vi "LEYBOLD.vi"() -> ()   [LabVIEW 2022 SP3]
uses:
  Enum/Enum p1.ctl
  <vilib>/Instr/_visa.llb/VISA Flush IO Buffer Mask.ctl
  Variables globales/Variable glob Leybold.vi
  Variables globales/Variable glob generale.vi
  <vilib>/Instr/_visa.llb/VISA Configure Serial Port (Instr).vi
panel:
  out "Données Leybold":string[](array[string])
  out "VISA":refnum<visa-resource-name>[](array[refnum])
  out "Chaine lue :":string
  # "Dialogue avec les CENTER-ONE"
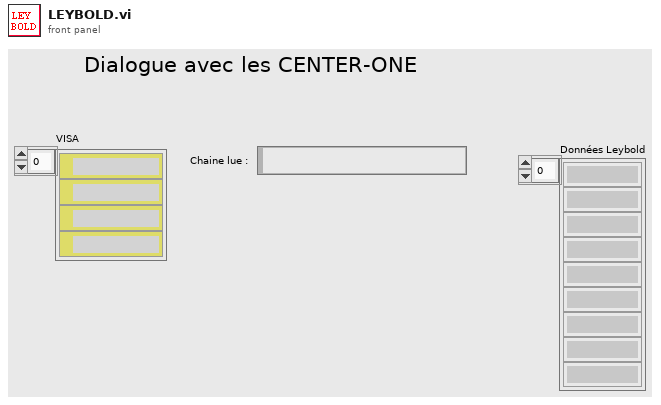
[diagram p1: front panel]
types:
  T1 = typedef "Enum p1.ctl" = enum16{"init", "Lecture pour vider buffer", "écriture val pres", "lecture ACK", "écriture ENQ", "lecture pres", "traitement chaine", "erreur"}
  T2 = typedef "VISA Flush IO Buffer Mask.ctl" = u16
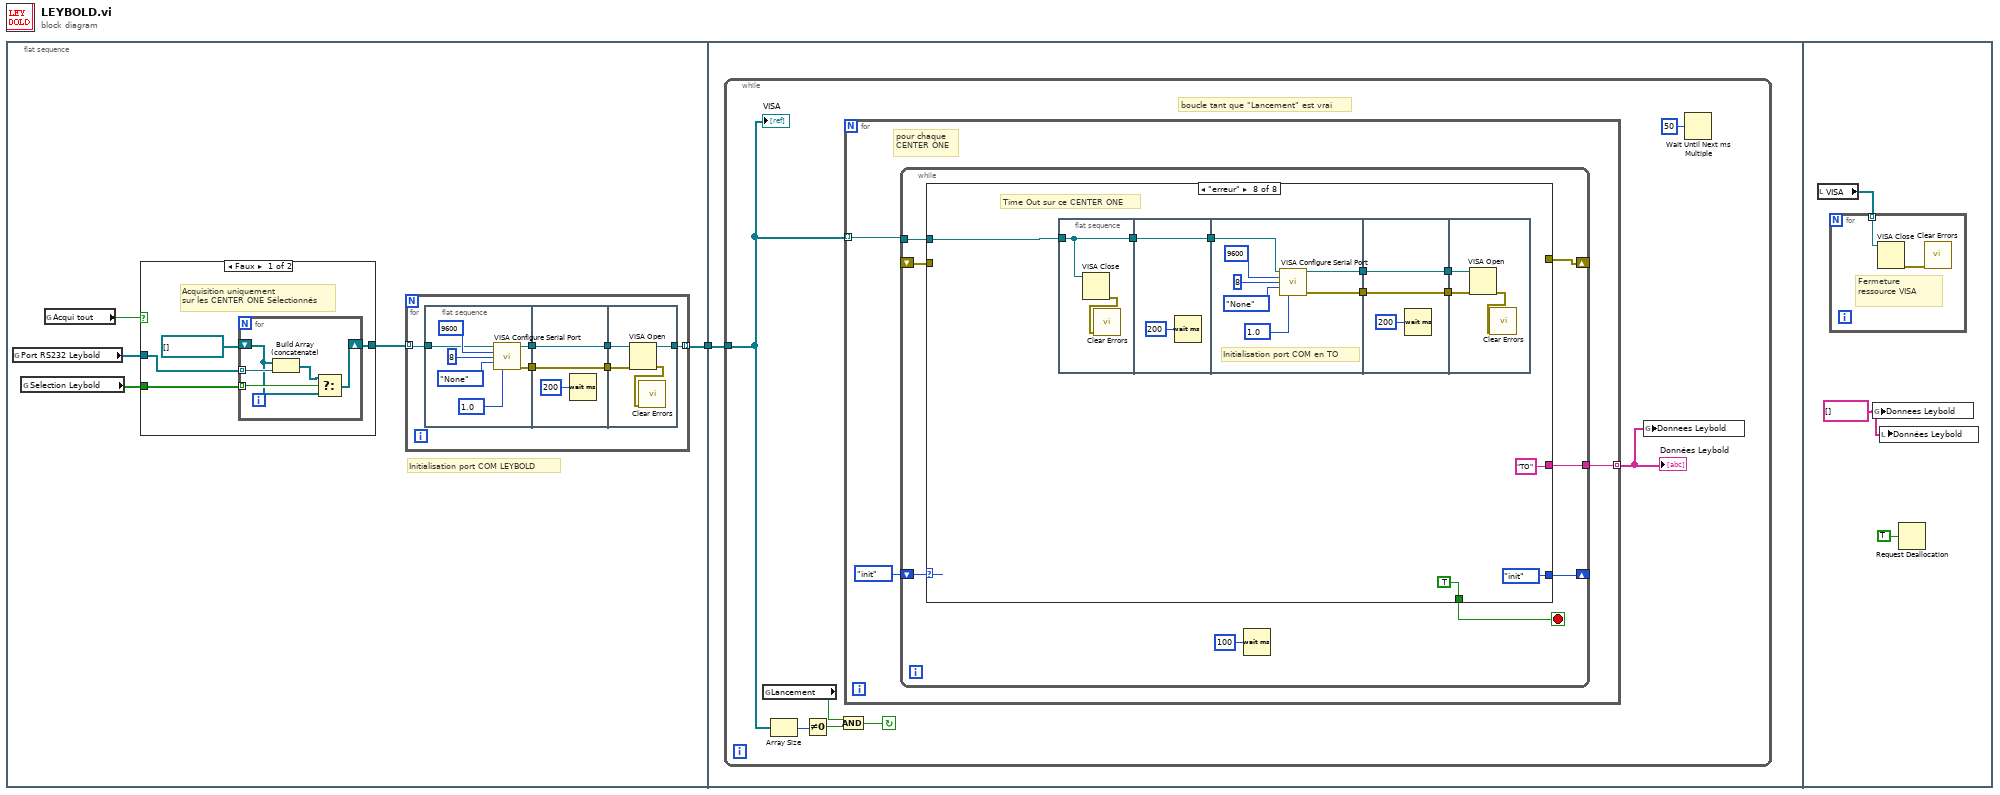
[diagram p0: block diagram]
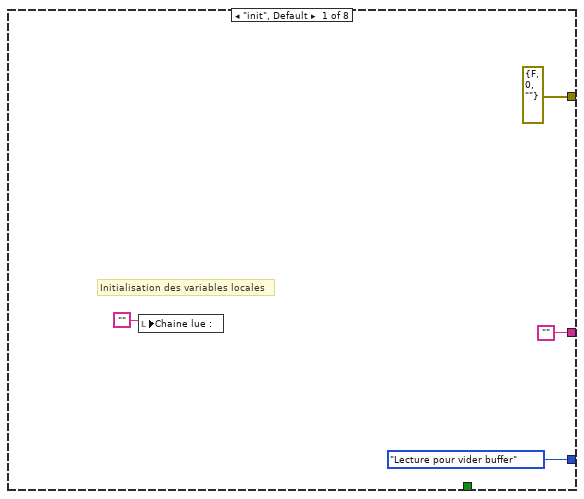
[diagram p3: hidden frame]
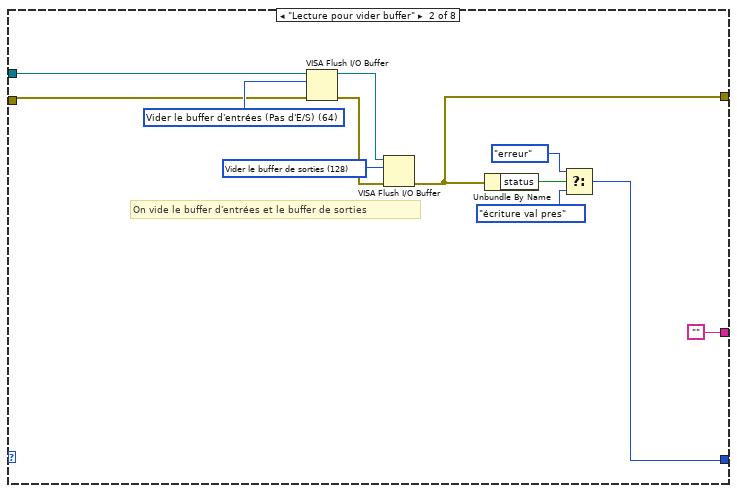
[diagram p4: hidden frame]
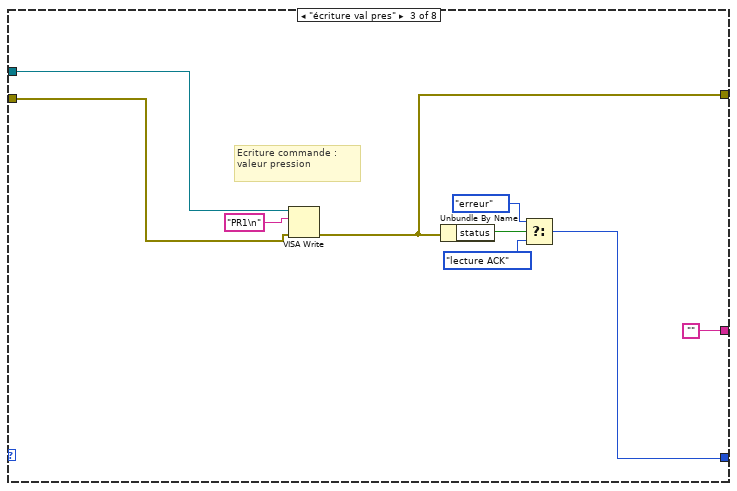
[diagram p5: hidden frame]
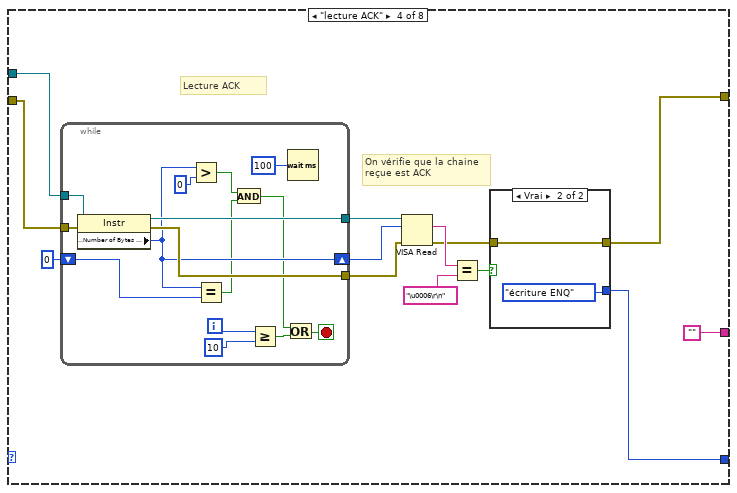
[diagram p6: hidden frame]
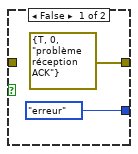
[diagram p7: hidden frame]
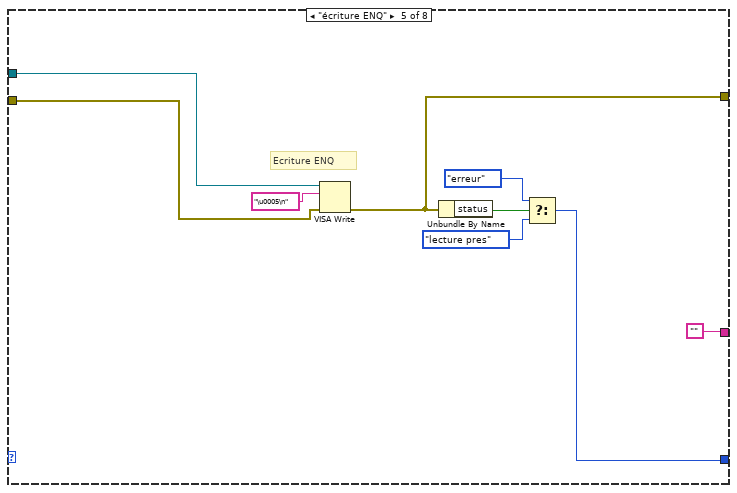
[diagram p8: hidden frame]
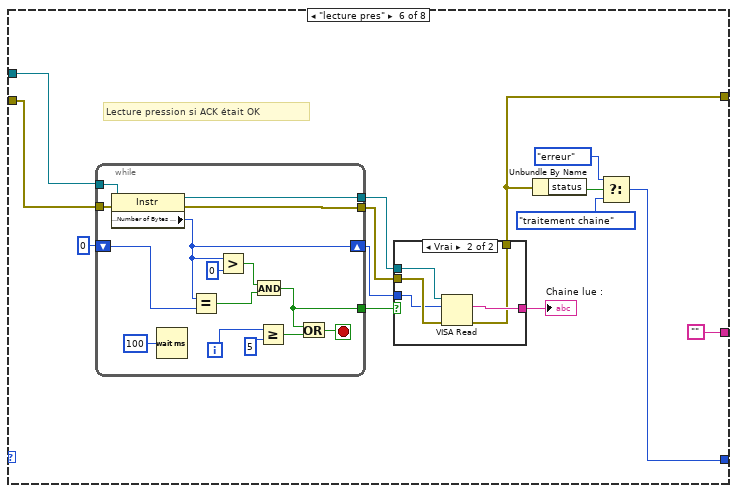
[diagram p9: hidden frame]
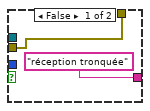
[diagram p10: hidden frame]
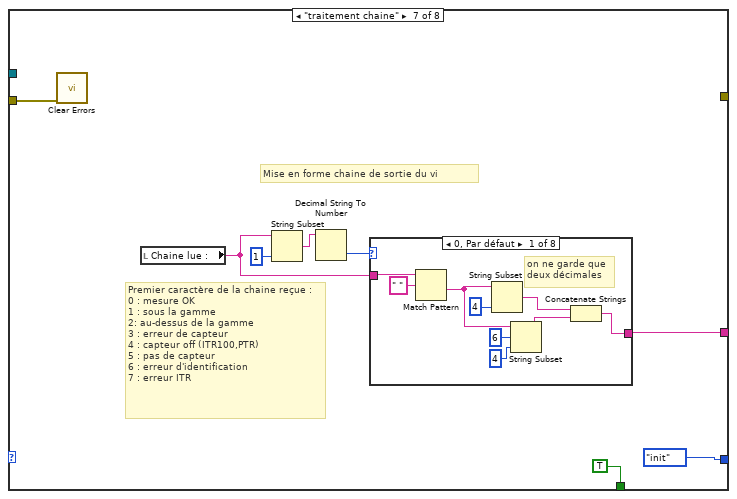
[diagram p11: hidden frame]
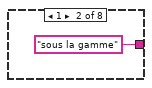
[diagram p12: hidden frame]
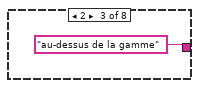
[diagram p13: hidden frame]
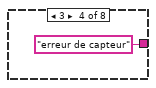
[diagram p14: hidden frame]
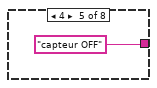
[diagram p15: hidden frame]
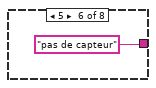
[diagram p16: hidden frame]
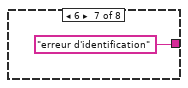
[diagram p17: hidden frame]
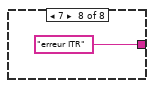
[diagram p18: hidden frame]
diagram:
  n1 = flat-sequence {
    tunnel: [w2] -> w1
    tunnel: w1 -> [w37]
    frame #0 {
      # "Initialisation port COM LEYBOLD"
      n2 = global read "Variable glob Leybold.vi" "Port RS232 Leybold"() -> (w4:refnum<visa-resource-name>[])
      n3 = global read "Variable glob Leybold.vi" "Selection Leybold"() -> (w3:bool[])
      n4 = global read "Variable glob generale.vi" "Acqui tout"() -> (w5:bool)
      n5 = case shown="Faux" w5 {
        tunnel: [w8 w16] -> w6
        tunnel: w4 -> [w10 w16]
        tunnel: w3 -> [w9 _]
        frame False {
          # "Acquisition uniquement\nsur les CENTER ONE Sélectionnés"
          n6 = for {
            tunnel: w10 -> [w14] mode=indexing
            tunnel: w9 -> [w15] mode=indexing
            shift-right: [w12] -> w8
            shift-left: refnum<visa-resource-name>[] [] -> [w11]
            n7 = Build Array (concatenate)(w11, w14) -> (w13:refnum<visa-resource-name>[])
            n8 = Select(t=w13, s=w15, f=w11) -> (s? t:f=w12:refnum<visa-resource-name>[])
          }
        }
        frame True {
          # "Acquisition sur l'ensemble\ndes CENTER ONE configurés"
        }
      }
      n9 = for {
        tunnel: w6 -> [w22] mode=indexing
        tunnel: [w19] -> w2 mode=indexing
        n10 = flat-sequence {
          tunnel: w22 -> [w25]
          tunnel: [w24] -> w21
          tunnel: [w23] -> w17
          tunnel: w21 -> [w31]
          tunnel: [w31] -> w20
          tunnel: [w30] -> w18
          tunnel: w17 -> [w30]
          tunnel: w20 -> [w36]
          tunnel: [w35] -> w19
          tunnel: w18 -> [w34]
          frame #0 {
            w29 = u16 10 items=["1.0"=10, "1.5"=15, "2.0"=20] ("stop bits (10: 1 bit)")
            n11 = call-poly "VISA Configure Serial Port"("VISA resource name"=w25, "baud rate (9600)"=u32 9600, "data bits (8)"=u16 8, "parity (0:none)"=enum16{"None", "Odd", "Even", "Mark", "Space"}."None", "stop bits (10: 1 bit)"=w29) -> ("VISA resource name out"=w24:refnum<visa-resource-name>, "error out"=w23:errorcluster)  [unwired: 9 in]
          }
          frame #1 {
            n12 = Wait (ms)(milliseconds to wait=u32 200 ("attente (ms)")) -> ()  [unwired: 1 out]
          }
          frame #2 {
            n13 = VISA Open(error in (no error)=w34, VISA resource name=w36) -> (VISA resource name=w35:refnum<visa-resource-name>, error out=w33:errorcluster)  [unwired: 3 in]
            n14 = call <vilib>:"Clear Errors.vi"("error in (no error)"=w33) -> ()  [unwired: 5 in, 2 out]
          }
        }
      }
    }
    frame #1 {
      n15 = while {
        tunnel: w37 -> [w42]
        stop <- w38 continue-if-true
        # "boucle tant que \"Lancement\" est vrai"
        n16 = global read "Variable glob generale.vi" "Lancement"() -> (w40:bool)
        n17 = Array Size(array=w42) -> (size(s)=w41:i32)
        n18 = Not Equal To 0?(x=w41) -> (x != 0?=w39:bool)
        n19 = And(x=w40, y=w39) -> (x .and. y?=w38:bool)
        n20 = for {
          tunnel: w42 -> [w46] mode=indexing
          tunnel: [w45] -> w43 mode=indexing
          # "pour chaque\nCENTER ONE"
          n21 = while {
            shift-right: [w53] -> _
            shift-left: Enum_p1."init" ("Énum") -> [w55]
            tunnel: [w52] -> w45
            tunnel: w46 -> [w54]
            shift-right: [w49] -> _
            shift-left: _ -> [w48]
            stop <- w51 stop-if-true
            n22 = case shown="\"erreur\"" w55 {
              tunnel: w54 -> [_ w71 w79 w89 w120 w134 _ w189]
              tunnel: [Enum_p1."Lecture pour vider buffer" ("Énum") w68 w76 w83 w115 w124 Enum_p1."init" ("Énum") Enum_p1."init" ("Énum")] -> w53
              tunnel: ["" "" "" "" "" "" w161 "TO"] -> w52
              tunnel: [_ _ _ _ _ _ TRUE TRUE] -> w51
              tunnel: [errorcluster {"status"=FALSE, "code"=0, "source"=""} ("error out") w70 w78 w84 w119 w128 _ _] -> w49
              tunnel: w48 -> [_ w61 w73 w82 w114 w123 w158 _]
              frame "init", Default {
                # "Initialisation des variables locales"
                n23 = local write "Chaine lue :"("") -> ()
              }
              frame "Lecture pour vider buffer" {
                w63 = T2 128 items=["Vider le buffer d'entrées"=16, "Écrire le buffer de sorties sur le périphérique"=32, "Vider le buffer d'entrées (Pas d'E/S)"=64, "Vider le buffer de sorties"=128] ("Mask")
                w65 = T2 64 items=["Vider le buffer d'entrées"=16, "Écrire le buffer de sorties sur le périphérique"=32, "Vider le buffer d'entrées (Pas d'E/S)"=64, "Vider le buffer de sorties"=128] ("Mask")
                # "On vide le buffer d'entrées et le buffer de sorties"
                n24 = VISA Flush I/O Buffer(VISA resource name=w71, mask (16)=w65, error in (no error)=w61) -> (VISA resource name out=w64:refnum<visa-resource-name>, error out=w62:errorcluster)
                n25 = VISA Flush I/O Buffer(VISA resource name=w64, mask (16)=w63, error in (no error)=w62) -> (error out=w70:errorcluster)  [unwired: 1 out]
                n26 = Unbundle By Name(w70) -> ("status"=w69:bool)
                n27 = Select(t=Enum_p1."erreur" ("Énum"), s=w69, f=Enum_p1."écriture val pres" ("Énum")) -> (s? t:f=w68:T1)
              }
              frame "écriture val pres" {
                # "Ecriture commande :\nvaleur pression"
                n28 = VISA Write(VISA resource name=w79, write buffer="PR1\n", error in (no error)=w73) -> (error out=w78:errorcluster)  [unwired: 2 out]
                n29 = Unbundle By Name(w78) -> ("status"=w77:bool)
                n30 = Select(t=Enum_p1."erreur" ("Énum"), s=w77, f=Enum_p1."lecture ACK" ("Énum")) -> (s? t:f=w76:T1)
              }
              frame "lecture ACK" {
                # "On vérifie que la chaine\nreçue est ACK"
                # "Lecture ACK"
                n31 = while {
                  tunnel: w89 -> [w112]
                  tunnel: [w108] -> w90
                  tunnel: [w107] -> w91
                  shift-right: [w103] -> w92
                  shift-left: 0 -> [w102]
                  tunnel: w82 -> [w98]
                  i -> [w111]
                  stop <- w105 stop-if-true
                  n32 = property class="Instr"(reference=w112, error in=w98) -> (reference out=w108:refnum<visa-resource-name>, error out=w107:errorcluster, "Serial Settings:Number of Bytes at Serial Port"=w103:u32)
                  n33 = Greater?(x=w103, y=u32 0) -> (0:w101:bool)
                  n34 = Equal?(x=w103, y=w102) -> (x = y?=w100:bool)
                  n35 = And(x=w101, y=w100) -> (x .and. y?=w99:bool)
                  n36 = Greater Or Equal?(x=w111, y=10) -> (x >= y?=w106:bool)
                  n37 = Or(x=w99, y=w106) -> (x .or. y?=w105:bool)
                  n38 = Wait (ms)(milliseconds to wait=u32 100 ("attente (ms)")) -> ()  [unwired: 1 out]
                }
                n39 = VISA Read(VISA resource name=w90, byte count=w92, error in (no error)=w91) -> (read buffer=w87:string, error out=w85:errorcluster)  [unwired: 2 out]
                n40 = Equal?(x=w87, y="\u0006\r\n") -> (x = y?=w86:bool)
                n41 = case shown="Vrai" w86 {
                  tunnel: w85 -> [_ w97]
                  tunnel: [errorcluster {"status"=TRUE, "code"=0, "source"="problème réception ACK"} ("error out") w97] -> w84
                  tunnel: [Enum_p1."erreur" ("Énum") Enum_p1."écriture ENQ" ("Énum")] -> w83
                  frame False {
                  }
                  frame True {
                  }
                }
              }
              frame "écriture ENQ" {
                # "Ecriture ENQ"
                n42 = VISA Write(VISA resource name=w120, write buffer="\u0005\n", error in (no error)=w114) -> (error out=w119:errorcluster)  [unwired: 2 out]
                n43 = Unbundle By Name(w119) -> ("status"=w118:bool)
                n44 = Select(t=Enum_p1."erreur" ("Énum"), s=w118, f=Enum_p1."lecture pres" ("Énum")) -> (s? t:f=w115:T1)
              }
              frame "lecture pres" {
                # "Lecture pression si ACK était OK"
                n45 = while {
                  tunnel: w134 -> [w157]
                  tunnel: [w144] -> w135
                  tunnel: [w151] -> w132
                  tunnel: [w150] -> w131
                  shift-right: [w148] -> w130
                  shift-left: 0 -> [w147]
                  tunnel: w123 -> [w143]
                  i -> [w155]
                  stop <- w153 stop-if-true
                  n46 = property class="Instr"(reference=w157, error in=w143) -> (reference out=w151:refnum<visa-resource-name>, error out=w150:errorcluster, "Serial Settings:Number of Bytes at Serial Port"=w148:u32)
                  n47 = Wait (ms)(milliseconds to wait=u32 100 ("attente (ms)")) -> ()  [unwired: 1 out]
                  n48 = Equal?(x=w148, y=w147) -> (x = y?=w145:bool)
                  n49 = Greater?(x=w148, y=u32 0) -> (0:w146:bool)
                  n50 = And(x=w146, y=w145) -> (x .and. y?=w144:bool)
                  n51 = Greater Or Equal?(x=w155, y=5) -> (x >= y?=w152:bool)
                  n52 = Or(x=w144, y=w152) -> (x .or. y?=w153:bool)
                }
                n53 = case shown="Vrai" w135 {
                  tunnel: w132 -> [_ w142]
                  tunnel: w131 -> [w136 w141]
                  tunnel: w130 -> [_ w140]
                  tunnel: ["réception tronquée" w139] -> w133
                  tunnel: [w136 w138] -> w128
                  frame False {
                  }
                  frame True {
                    n54 = VISA Read(VISA resource name=w142, byte count=w140, error in (no error)=w141) -> (read buffer=w139:string, error out=w138:errorcluster)  [unwired: 2 out]
                  }
                }
                "Chaine lue :" <- w133
                n55 = Unbundle By Name(w128) -> ("status"=w126:bool)
                n56 = Select(t=Enum_p1."erreur" ("Énum"), s=w126, f=Enum_p1."traitement chaine" ("Énum")) -> (s? t:f=w124:T1)
              }
              frame "traitement chaine" {
                # "Premier caractère de la chaine reçue :\n0 : mesure OK\n1 : sous la gamme\n2: au-dessus de la gamme\n3 : erreur de capteur\n4 : capteur off (ITR100,PTR)\n5 : pas de capteur\n6 : erreur d'identification\n7 : erreur ITR"
                # "Mise en forme chaine de sortie du vi"
                n57 = call <vilib>:"Clear Errors.vi"("error in (no error)"=w158) -> ()  [unwired: 5 in, 2 out]
                n58 = local read "Chaine lue :"() -> (w165:string)
                n59 = String Subset(string=w165, length (rest)=1 ("longueur (reste)")) -> (substring=w164:string)  [unwired: 1 in]
                n60 = Decimal String To Number(string=w164) -> (number=w162:i32)  [unwired: 2 in, 1 out]
                n61 = case shown="0, Par défaut" w162 {
                  tunnel: [w173 "sous la gamme" "au-dessus de la gamme" "erreur de capteur" "capteur OFF" "pas de capteur" "erreur d'identification" "erreur ITR"] -> w161
                  tunnel: w165 -> [w172 _ _ _ _ _ _ _]
                  frame 0, Default {
                    # "on ne garde que\ndeux décimales"
                    n62 = Match Pattern(string=w172, regular expression=" " ("expression")) -> (after substring=w170:string)  [unwired: 1 in, 3 out]
                    n63 = String Subset(string=w170, length (rest)=4 ("longueur (reste)")) -> (substring=w168:string)  [unwired: 1 in]
                    n64 = String Subset(string=w170, offset (0)=6, length (rest)=4 ("longueur (reste)")) -> (substring=w167:string)
                    n65 = Concatenate Strings(w168, w167) -> (w173:string)
                  }
                  frame 1 {
                  }
                  frame 2 {
                  }
                  frame 3 {
                  }
                  frame 4 {
                  }
                  frame 5 {
                  }
                  frame 6 {
                  }
                  frame 7 {
                  }
                }
              }
              frame "erreur" {
                # "Time Out sur ce CENTER ONE"
                n66 = flat-sequence {
                  tunnel: w189 -> [w193]
                  tunnel: [w193] -> w187
                  tunnel: [w194] -> w188
                  tunnel: w187 -> [w194]
                  tunnel: w188 -> [w198]
                  tunnel: [w197] -> w185
                  tunnel: [w196] -> w184
                  tunnel: [w204] -> w186
                  tunnel: w185 -> [w204]
                  tunnel: w184 -> [w203]
                  tunnel: [w203] -> w183
                  tunnel: w186 -> [w208]
                  tunnel: w183 -> [w207]
                  frame #0 {
                    n67 = VISA Close(VISA resource name=w193) -> (error out=w192:errorcluster)  [unwired: 1 in]
                    n68 = call <vilib>:"Clear Errors.vi"("error in (no error)"=w192) -> ()  [unwired: 5 in, 2 out]
                  }
                  frame #1 {
                    n69 = Wait (ms)(milliseconds to wait=u32 200 ("attente (ms)")) -> ()  [unwired: 1 out]
                  }
                  frame #2 {
                    w202 = u16 10 items=["1.0"=10, "1.5"=15, "2.0"=20] ("stop bits (10: 1 bit)")
                    # "Initialisation port COM en TO"
                    n70 = call-poly "VISA Configure Serial Port"("VISA resource name"=w198, "baud rate (9600)"=u32 9600, "data bits (8)"=u16 8, "parity (0:none)"=enum16{"None", "Odd", "Even", "Mark", "Space"}."None", "stop bits (10: 1 bit)"=w202) -> ("VISA resource name out"=w196:refnum<visa-resource-name>, "error out"=w197:errorcluster)  [unwired: 9 in]
                  }
                  frame #3 {
                    n71 = Wait (ms)(milliseconds to wait=u32 200 ("attente (ms)")) -> ()  [unwired: 1 out]
                  }
                  frame #4 {
                    n72 = VISA Open(error in (no error)=w208, VISA resource name=w207) -> (error out=w206:errorcluster)  [unwired: 3 in, 1 out]
                    n73 = call <vilib>:"Clear Errors.vi"("error in (no error)"=w206) -> ()  [unwired: 5 in, 2 out]
                  }
                }
              }
            }
            n74 = Wait (ms)(milliseconds to wait=u32 100 ("attente (ms)")) -> ()  [unwired: 1 out]
          }
        }
        "Données Leybold" <- w43
        n75 = global write "Variable glob Leybold.vi" "Donnees Leybold"(w43) -> ()
        n76 = Wait Until Next ms Multiple(millisecond multiple=u32 50 ("n millisecondes")) -> ()  [unwired: 1 out]
        "VISA" <- w42
      }
    }
    frame #2 {
      w209 = string[] [] ("Données Leybold")
      n77 = local read "VISA"() -> (w210:refnum<visa-resource-name>[])
      n78 = for {
        tunnel: w210 -> [w212] mode=indexing
        # "Fermeture\nressource VISA"
        n79 = VISA Close(VISA resource name=w212) -> (error out=w213:errorcluster)  [unwired: 1 in]
        n80 = call <vilib>:"Clear Errors.vi"("error in (no error)"=w213) -> ()  [unwired: 5 in, 2 out]
      }
      n81 = global write "Variable glob Leybold.vi" "Donnees Leybold"(w209) -> ()
      n82 = local write "Données Leybold"(w209) -> ()
      n83 = Request Deallocation(TRUE ("flag")) -> ()
    }
  }
